vi "power_measure.vi"(10 "Stop Refnum":refnum<vi>, 11 "Measured Power Refnum":refnum<vi>) -> ()   [LabVIEW 2025, in "tSNIP.lvlib"]
uses:
  tSNIP.lvlib
panel:
  out "Power (W)":dbl(graph)=-5.8e-06
  in  "OphirLMMeasurementLib.ICoLMMeasurement2":refnum<k7>
  out "error out":errorcluster
  in  "error in":errorcluster
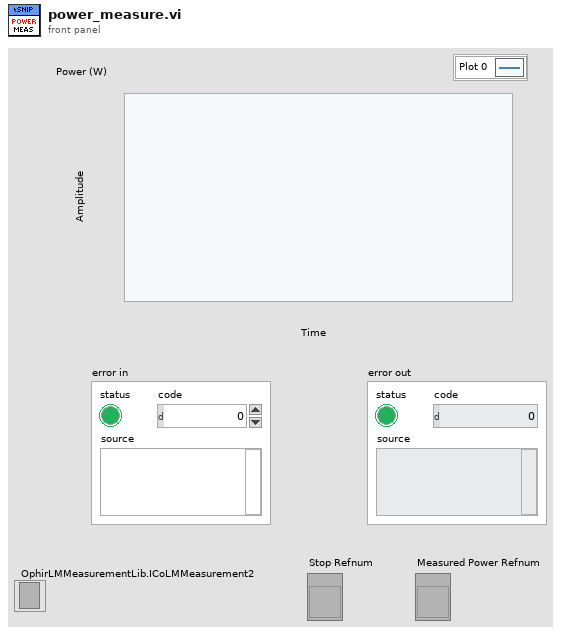
[diagram p1: front panel]
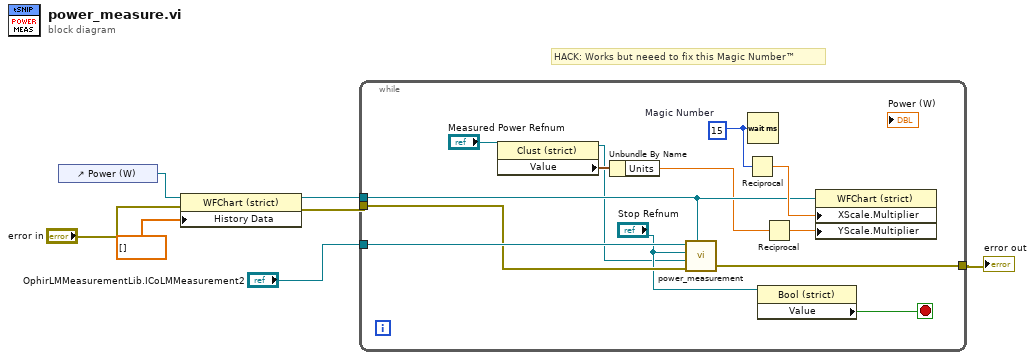
[diagram p0: block diagram]
diagram:
  # "HACK: Works but neeed to fix this Magic Number™"
  n1 = control-ref of="Power (W)"() -> (w6:refnum<vi>)
  n2 = property class="WFChart (strict)"(reference=w6, error in="error in", "History Data"=dbl[] []) -> (reference out=w3:refnum<vi>, error out=w2:errorcluster)
  n3 = while {
    tunnel: "OphirLMMeasurementLib.ICoLMMeasurement2" -> [w20]
    tunnel: [w19] -> w1
    tunnel: w3 -> [w16]
    tunnel: w2 -> [w15]
    stop <- w13 stop-if-true
    w17 = u32 15  # Magic Number
    n4 = property class="Clust (strict)"(reference="Measured Power Refnum") -> (reference out=w8:refnum<vi>, "Value"=w10:cluster{"Value":dbl, "Units":dbl})  [unwired: 1 in, 1 out]
    n5 = Unbundle By Name(w10) -> ("Units"=w9:dbl)
    n6 = call "power_measurement.vi"("Measured Power Chart Ref"=w16, "error in"=w15, "Measured Power Ref"=w8, "Stop Ref"="Stop Refnum", "OphirLMMeasurementLib.ICoLMMeasurement2"=w20) -> ("error out"=w19:errorcluster)  [unwired: 6 in]
    n7 = Reciprocal(x=w17) -> (1/x=w18:dbl)
    n8 = Wait (ms)(milliseconds to wait=w17) -> ()  [unwired: 1 out]
    n9 = property class="Bool (strict)"(reference="Stop Refnum") -> ("Value"=w13:bool)  [unwired: 1 in, 2 out]
    n10 = Reciprocal(x=w9) -> (1/x=w11:dbl)
    n11 = property class="WFChart (strict)"(reference=w16, "XScale.Multiplier"=w18, "YScale.Multiplier"=w11) -> ()  [unwired: 1 in, 2 out]
  }
  "error out" <- w1
